vi "PathPlanner_Cmd_AutoHolonomicExecute.vi"(5 "PathPlanner_Cmd_FollowHolConfig":T17={"HOLONOMIC_CTRL_PACK_TUNING"={"X PID Tuning"={"Kp"=0.0, "Ki"=0.0, "Kd"=0.0, "MaximumIntegral"=9.9e+30, "MinimumIntegral"=-9.9e+30, "IntegralZone"=9.9e+30}, "Y PID Tuning"={"Kp"=0.0, "Ki"=0.0, "Kd"=0.0, "MaximumIntegral"=9.9e+30, "MinimumIntegral"=-9.9e+30, "IntegralZone"=9.9e+30}, "thetaProfiledPID_CTRL"={"Controller"={"Kp"=0.0, "Ki"=0.0, "Kd"=0.0, "Period"=0.0, "Max_Integral"=1.0, "Min_Integral"=-1.0, "Max_Input"=0.0, "Min_Input"=0.0, "Continuous"=FALSE, "PositionError"=0.0, "VelocityError"=0.0, "PrevError"=0.0, "Total_Integral"=0.0, "PositionTolerance"=0.05, "VelocityTolerance"=9.99e+35, "SetPoint"=0.0, "Kf"=0.0, "Prev_Deriv"=0.0, "Prev_Deriv 2"=0.0, "DerivativeFilter"=FALSE, "Min_Output"=-9.99e+35, "Max_Output"=9.9e+35, "Prev_F_P"=0.0, "Prev_F_P_2"=0.0, "AntiWindupActive"=FALSE, "Measurement"=0.0, "IntegralZone"=9.9e+30}, "Goal"={"Position"=0.0, "Velocity"=0.0}, "Setpoint"={"Position"=0.0, "Velocity"=0.0}, "Constraint"={"MaxVelocity"=0.0, "MaxAcceleration"=0.0}}}, "Max Wheel Speed M/S"=0.0, "Tolerance SI"={"TRANSLATION"={"X"=0.04, "Y"=0.04}, "ROTATION"={"VALUE"=0.034906585039887, "COS"=0.999390827019096, "SIN"=0.034899496702501}}, "Drive Base Radius M"=0.0, "ControlPastEnd_Sec"=3.0, "Period_Sec"=0.02, "Trigger Events"=TRUE} {"Tolerance SI"."ROTATION"."SIN" format="%13.4f"; "Tolerance SI"."ROTATION"."COS" format="%13.4f"; "Tolerance SI"."ROTATION"."VALUE" format="%13.4f"; "Tolerance SI"."TRANSLATION"."Y" format="%14.3f"; "Tolerance SI"."TRANSLATION"."X" format="%14.3f"; "HOLONOMIC_CTRL_PACK_TUNING"."thetaProfiledPID_CTRL"."Constraint"."MaxAcceleration" format="%16_6e"; "HOLONOMIC_CTRL_PACK_TUNING"."thetaProfiledPID_CTRL"."Constraint"."MaxVelocity" format="%16_6e"; "HOLONOMIC_CTRL_PACK_TUNING"."thetaProfiledPID_CTRL"."Setpoint"."Velocity" format="%16_6e"; "HOLONOMIC_CTRL_PACK_TUNING"."thetaProfiledPID_CTRL"."Setpoint"."Position" format="%16_6e"; "HOLONOMIC_CTRL_PACK_TUNING"."thetaProfiledPID_CTRL"."Goal"."Velocity" format="%16_6e"; "HOLONOMIC_CTRL_PACK_TUNING"."thetaProfiledPID_CTRL"."Goal"."Position" format="%16_6e"; "HOLONOMIC_CTRL_PACK_TUNING"."thetaProfiledPID_CTRL"."Controller"."IntegralZone" format="%16_6e"; "HOLONOMIC_CTRL_PACK_TUNING"."thetaProfiledPID_CTRL"."Controller"."Measurement" format="%16_6e"; "HOLONOMIC_CTRL_PACK_TUNING"."thetaProfiledPID_CTRL"."Controller"."Prev_F_P_2" format="%16_6e"; "HOLONOMIC_CTRL_PACK_TUNING"."thetaProfiledPID_CTRL"."Controller"."Prev_F_P" format="%16_6e"; "HOLONOMIC_CTRL_PACK_TUNING"."thetaProfiledPID_CTRL"."Controller"."Max_Output" format="%16_6e"; "HOLONOMIC_CTRL_PACK_TUNING"."thetaProfiledPID_CTRL"."Controller"."Min_Output" format="%16_6e"; "HOLONOMIC_CTRL_PACK_TUNING"."thetaProfiledPID_CTRL"."Controller"."Prev_Deriv 2" format="%16_6e"; "HOLONOMIC_CTRL_PACK_TUNING"."thetaProfiledPID_CTRL"."Controller"."Prev_Deriv" format="%16_6e"; "HOLONOMIC_CTRL_PACK_TUNING"."thetaProfiledPID_CTRL"."Controller"."Kf" format="%16_6e"; "HOLONOMIC_CTRL_PACK_TUNING"."thetaProfiledPID_CTRL"."Controller"."SetPoint" format="%16_6e"; "HOLONOMIC_CTRL_PACK_TUNING"."thetaProfiledPID_CTRL"."Controller"."VelocityTolerance" format="%16_6e"; "HOLONOMIC_CTRL_PACK_TUNING"."thetaProfiledPID_CTRL"."Controller"."PositionTolerance" format="%16_6e"; "HOLONOMIC_CTRL_PACK_TUNING"."thetaProfiledPID_CTRL"."Controller"."Total_Integral" format="%16_6e"; "HOLONOMIC_CTRL_PACK_TUNING"."thetaProfiledPID_CTRL"."Controller"."PrevError" format="%16_6e"; "HOLONOMIC_CTRL_PACK_TUNING"."thetaProfiledPID_CTRL"."Controller"."VelocityError" format="%16_6e"; "HOLONOMIC_CTRL_PACK_TUNING"."thetaProfiledPID_CTRL"."Controller"."PositionError" format="%16_6e"; "HOLONOMIC_CTRL_PACK_TUNING"."thetaProfiledPID_CTRL"."Controller"."Min_Input" format="%16_6e"; "HOLONOMIC_CTRL_PACK_TUNING"."thetaProfiledPID_CTRL"."Controller"."Max_Input" format="%16_6e"; "HOLONOMIC_CTRL_PACK_TUNING"."thetaProfiledPID_CTRL"."Controller"."Min_Integral" format="%16_6e"; "HOLONOMIC_CTRL_PACK_TUNING"."thetaProfiledPID_CTRL"."Controller"."Max_Integral" format="%16_6e"; "HOLONOMIC_CTRL_PACK_TUNING"."thetaProfiledPID_CTRL"."Controller"."Period" format="%16_6e"; "HOLONOMIC_CTRL_PACK_TUNING"."thetaProfiledPID_CTRL"."Controller"."Kd" format="%16_6e"; "HOLONOMIC_CTRL_PACK_TUNING"."thetaProfiledPID_CTRL"."Controller"."Ki" format="%16_6e"; "HOLONOMIC_CTRL_PACK_TUNING"."thetaProfiledPID_CTRL"."Controller"."Kp" format="%16_6e"}, 6 "PassthroughTime_SEC":dbl=-1.0, 7 "PathPlanner_Cmd_AutoConfig":T2 {"Paths"."IdealStartingState"."Rotation"."SIN" format="%13.4f"; "Paths"."IdealStartingState"."Rotation"."COS" format="%13.4f"; "Paths"."IdealStartingState"."Rotation"."VALUE" format="%13.4f"; "Paths"."PointTowardsZones"."TargetPosition"."Y" format="%14.3f"; "Paths"."PointTowardsZones"."TargetPosition"."X" format="%14.3f"; "Paths"."PointTowardsZones"."RotationOffset"."SIN" format="%13.4f"; "Paths"."PointTowardsZones"."RotationOffset"."COS" format="%13.4f"; "Paths"."PointTowardsZones"."RotationOffset"."VALUE" format="%13.4f"; "Paths"."Waypoints"."nextControl"."Y" format="%14.3f"; "Paths"."Waypoints"."nextControl"."X" format="%14.3f"; "Paths"."Waypoints"."anchor"."Y" format="%14.3f"; "Paths"."Waypoints"."anchor"."X" format="%14.3f"; "Paths"."Waypoints"."prevControl"."Y" format="%14.3f"; "Paths"."Waypoints"."prevControl"."X" format="%14.3f"; "Paths"."AllPoints"."RotationTarget"."rotation"."SIN" format="%13.4f"; "Paths"."AllPoints"."RotationTarget"."rotation"."COS" format="%13.4f"; "Paths"."AllPoints"."RotationTarget"."rotation"."VALUE" format="%13.4f"; "Paths"."AllPoints"."Position"."Y" format="%14.3f"; "Paths"."AllPoints"."Position"."X" format="%14.3f"; "Paths"."GoalEndState"."Rotation"."SIN" format="%13.4f"; "Paths"."GoalEndState"."Rotation"."COS" format="%13.4f"; "Paths"."GoalEndState"."Rotation"."VALUE" format="%13.4f"; "Paths"."RotationTargets"."rotation"."SIN" format="%13.4f"; "Paths"."RotationTargets"."rotation"."COS" format="%13.4f"; "Paths"."RotationTargets"."rotation"."VALUE" format="%13.4f"}, 8 "Enabled":bool=TRUE, 9 "Reset":bool, 10 "CurrentChassisSpeeds":T1 {"vOmega" format="%10.3f"; "vY" format="%10.3f"; "vX" format="%10.3f"}, 11 "Current Pose SI":T24={"TRANSLATION"={"X"=0.0, "Y"=0.0}, "ROTATION"={"VALUE"=0.0, "COS"=1.0, "SIN"=0.0}} {"ROTATION"."SIN" format="%13.4f"; "ROTATION"."COS" format="%13.4f"; "ROTATION"."VALUE" format="%13.4f"; "TRANSLATION"."Y" format="%14.3f"; "TRANSLATION"."X" format="%14.3f"}) -> (0 "Position Error M":dbl, 1 "Complete":bool, 2 "At Reference":bool, 3 "calcChassisSpeed":T1 {"vOmega" format="%10.3f"; "vY" format="%10.3f"; "vX" format="%10.3f"})   [LabVIEW 2019, in "PathPlanner24.lvlib"]
doc: "DOCUMENTATION IS NOT COMPLETE.\n \nCalculates the next output of the path following controller for holonomic drive robots. This wraps a Holonomic Drive Control function with the particulars needed to follow a PathPlanner trajectory.\n\nInputs:\n - PathPlanner_Holonomic_Ctrl_Pack_Tuning - cluster - The tuning paraameters for the holonomic drive controller. These are static. They should not be changed after the first call to this function.\n - CurrentPoseSi - pose2d - The current pose calculated by odometry or pose estimation. The pose can be absolute or relative depending on what type of trajectory is being followed.\n - PathPlannerState - cluster - The path palnner trajectory state containing the desired position and velocities of the robot.\n - Reset - boolean - When TRUE the holonomic drive controller is reset. This should be set to TRUE for the first execution of a trajectory.\n - Enabled - boolean - When TRUE, closed loop control is enabled. (Optional. Default: TRUE)\n - Period - double - The loop period in seconds for this controller. (Optional. Default: 0.020)\n\nOutputs:\n - CalcChassisSpeed - cluster - The desired chassis speed in SI units.\n - AtReference - boolean - TRUE if the robots position is within the defined tolerance.\n - PositionError - pose2d - Position error in SI units. How far the robot is away from the desired trajectory position.\n - out_Holonomic_Drive_Ctrl - THe current holonomic drive controller data cluster. This is mainly for diagnostic purposes."
uses:
  PathPlanner24.lvlib
  <vilib>/Rock Robotics/WPI/ThirdParty/JAS_Junk/TrajLib/TypeDef/CHASSIS_SPEEDS.ctl
  <vilib>/Rock Robotics/WPI/ThirdParty/JAS_Junk/TrajLib/Trajectory_Library.lvlib
  <vilib>/Rock Robotics/WPI/ThirdParty/JAS_Junk/TrajLib/TypeDef/TRANSLATION2D.ctl
  <vilib>/Rock Robotics/WPI/ThirdParty/JAS_Junk/TrajLib/TypeDef/ROTATION2D.ctl
  <vilib>/Rock Robotics/WPI/ThirdParty/JAS_Junk/TrajLib/TypeDef/POSE2D.ctl
  <vilib>/Rock Robotics/WPI/ThirdParty/JAS_Junk/TrajLib/TypeDef/PID_TUNING.ctl
  <vilib>/Rock Robotics/WPI/ThirdParty/JAS_Junk/TrajLib/TypeDef/PID_CONTROLLER.ctl
  <vilib>/Rock Robotics/WPI/ThirdParty/JAS_Junk/TrajLib/TypeDef/TRAPEZOID_PROFILE_STATE.ctl
  <vilib>/Rock Robotics/WPI/ThirdParty/JAS_Junk/TrajLib/TypeDef/TRAPEZOID_PROFILE_CONSTRAINT.ctl
  <vilib>/Rock Robotics/WPI/ThirdParty/JAS_Junk/TrajLib/TypeDef/PROFILED_PID_CONTROLLER.ctl
  <vilib>/Rock Robotics/WPI/ThirdParty/JAS_Junk/TrajLib/TypeDef/HOLONOMIC_PACK_TUNING.ctl
  TypeDef/PathPlannerRotationTarget.ctl
  TypeDef/PathPlannerPathConstraints.ctl
  TypeDef/PathPlannerConstraintsZone.ctl
  TypeDef/PathPlannerCommandUtil.ctl
  TypeDef/PathPlannerEventMarker.ctl
  TypeDef/PathPlannerGoalEndState.ctl
  TypeDef/PathPlannerPathPoint.ctl
  TypeDef/PathPlannerPath.ctl
  TypeDef/PathPlannerCmdFollowHolConfig.ctl
  TypeDef/PathPlannerWaypoint.ctl
  TypeDef/PathPlannerPointTowardsZone.ctl
  TypeDef/PathPlannerIdealStartingState.ctl
  TypeDef/PathPlannerCmdPathPlannerAutoConfig.ctl
  ENum/PathPlanner_CommandUtil_Type_ENUM.ctl
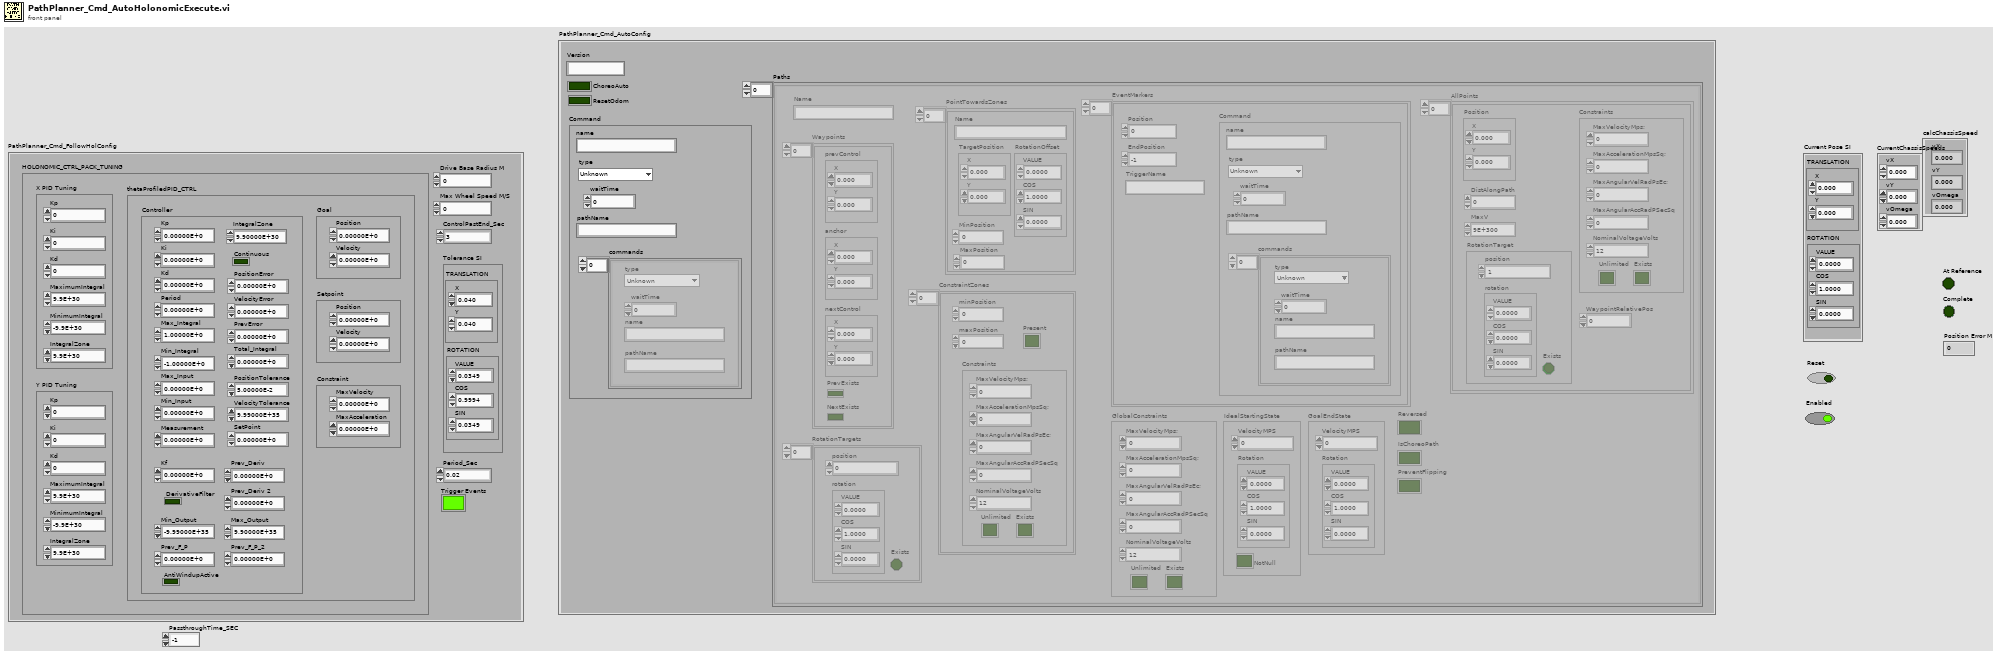
[diagram p1: front panel]
types:
  T1 = typedef "Trajectory_Library.lvlib/CHASSIS_SPEEDS.ctl" = cluster{"vX":dbl, "vY":dbl, "vOmega":dbl}
  T2 = typedef "PathPlanner24.lvlib/PathPlannerCmdPathPlannerAutoConfig.ctl" = cluster{"Command":T3, "ChoreoAuto":bool, "Version":string, "ResetOdom":bool, "Paths":T5[]}
  T3 = typedef "PathPlanner24.lvlib/PathPlannerCommandUtil.ctl" = cluster{"waitTime":dbl, "name":string, "pathName":string, "commands":cluster{"type":T4, "waitTime":dbl, "name":string, "pathName":string}[], "type":T4}
  T4 = typedef "PathPlanner24.lvlib/PathPlanner_CommandUtil_Type_ENUM.ctl" = enum16{"Unknown", "Wait", "Named", "Path", "Sequential", "Parallel", "Race", "Deadline", "PointTowardsZoneEnter", "PointTowardsZoneExit", "TriggerEventStart", "TriggerEventStop", "TriggerEventOneshot"}
  T5 = typedef "PathPlanner24.lvlib/PathPlannerPath.ctl" = cluster{"Reversed":bool, "RotationTargets":T6[], "ConstraintZones":T8[], "EventMarkers":T10[], "GlobalConstraints":T9, "GoalEndState":T11, "AllPoints":T12[], "Name":string, "Waypoints":T14[], "PointTowardsZones":T15[], "IdealStartingState":T16, "IsChoreoPath":bool, "PreventFlipping":bool}
  T6 = typedef "PathPlanner24.lvlib/PathPlannerRotationTarget.ctl" = cluster{"position":dbl, "rotation":T7, "Exists":bool}
  T7 = typedef "Trajectory_Library.lvlib/ROTATION2D.ctl" = cluster{"VALUE":dbl, "COS":dbl, "SIN":dbl}
  T8 = typedef "PathPlanner24.lvlib/PathPlannerConstraintsZone.ctl" = cluster{"minPosition":dbl, "maxPosition":dbl, "Constraints":T9, "Present":bool}
  T9 = typedef "PathPlanner24.lvlib/PathPlannerPathConstraints.ctl" = cluster{"MaxVelocityMps;":dbl, "MaxAccelerationMpsSq;":dbl, "MaxAngularVelRadPsEc;":dbl, "MaxAngularAccRadPSecSq":dbl, "Exists":bool, "Unlimited":bool, "NominalVoltageVolts":dbl}
  T10 = typedef "PathPlanner24.lvlib/PathPlannerEventMarker.ctl" = cluster{"Position":dbl, "Command":T3, "TriggerName":string, "EndPosition":dbl}
  T11 = typedef "PathPlanner24.lvlib/PathPlannerGoalEndState.ctl" = cluster{"VelocityMPS":dbl, "Rotation":T7}
  T12 = typedef "PathPlanner24.lvlib/PathPlannerPathPoint.ctl" = cluster{"Position":T13, "DistAlongPath":dbl, "MaxV":dbl, "Constraints":T9, "RotationTarget":T6, "WaypointRelativePos":dbl}
  T13 = typedef "Trajectory_Library.lvlib/TRANSLATION2D.ctl" = cluster{"X":dbl, "Y":dbl}
  T14 = typedef "PathPlanner24.lvlib/PathPlannerWaypoint.ctl" = cluster{"prevControl":T13, "anchor":T13, "nextControl":T13, "PrevExists":bool, "NextExists":bool}
  T15 = typedef "PathPlanner24.lvlib/PathPlannerPointTowardsZone.ctl" = cluster{"RotationOffset":T7, "Name":string, "TargetPosition":T13, "MinPosition":dbl, "MaxPosition":dbl}
  T16 = typedef "PathPlanner24.lvlib/PathPlannerIdealStartingState.ctl" = cluster{"VelocityMPS":dbl, "Rotation":T7, "NotNull":bool}
  T17 = typedef "PathPlanner24.lvlib/PathPlannerCmdFollowHolConfig.ctl" = cluster{"HOLONOMIC_CTRL_PACK_TUNING":T18, "Max Wheel Speed M/S":dbl, "Tolerance SI":T24, "Drive Base Radius M":dbl, "ControlPastEnd_Sec":dbl, "Period_Sec":dbl, "Trigger Events":bool}
  T18 = typedef "Trajectory_Library.lvlib/HOLONOMIC_PACK_TUNING.ctl" = cluster{"X PID Tuning":T19, "Y PID Tuning":T19, "thetaProfiledPID_CTRL":T20}
  T19 = typedef "Trajectory_Library.lvlib/PID_TUNING.ctl" = cluster{"Kp":dbl, "Ki":dbl, "Kd":dbl, "MaximumIntegral":dbl, "MinimumIntegral":dbl, "IntegralZone":dbl}
  T20 = typedef "Trajectory_Library.lvlib/PROFILED_PID_CONTROLLER.ctl" = cluster{"Controller":T21, "Goal":T22, "Setpoint":T22, "Constraint":T23}
  T21 = typedef "Trajectory_Library.lvlib/PID_CONTROLLER.ctl" = cluster{"Kp":dbl, "Ki":dbl, "Kd":dbl, "Period":dbl, "Max_Integral":dbl, "Min_Integral":dbl, "Max_Input":dbl, "Min_Input":dbl, "Continuous":bool, "PositionError":dbl, "VelocityError":dbl, "PrevError":dbl, "Total_Integral":dbl, "PositionTolerance":dbl, "VelocityTolerance":dbl, "SetPoint":dbl, "Kf":dbl, "Prev_Deriv":dbl, "Prev_Deriv 2":dbl, "DerivativeFilter":bool, "Min_Output":dbl, "Max_Output":dbl, "Prev_F_P":dbl, "Prev_F_P_2":dbl, "AntiWindupActive":bool, "Measurement":dbl, "IntegralZone":dbl}
  T22 = typedef "Trajectory_Library.lvlib/TRAPEZOID_PROFILE_STATE.ctl" = cluster{"Position":dbl, "Velocity":dbl}
  T23 = typedef "Trajectory_Library.lvlib/TRAPEZOID_PROFILE_CONSTRAINT.ctl" = cluster{"MaxVelocity":dbl, "MaxAcceleration":dbl}
  T24 = typedef "Trajectory_Library.lvlib/POSE2D.ctl" = cluster{"TRANSLATION":T13, "ROTATION":T7}
  T25 = cluster{"type":T4, "waitTime":dbl, "name":string, "pathName":string}[]
  T26 = cluster{"type":T4, "waitTime":dbl, "name":string, "pathName":string}
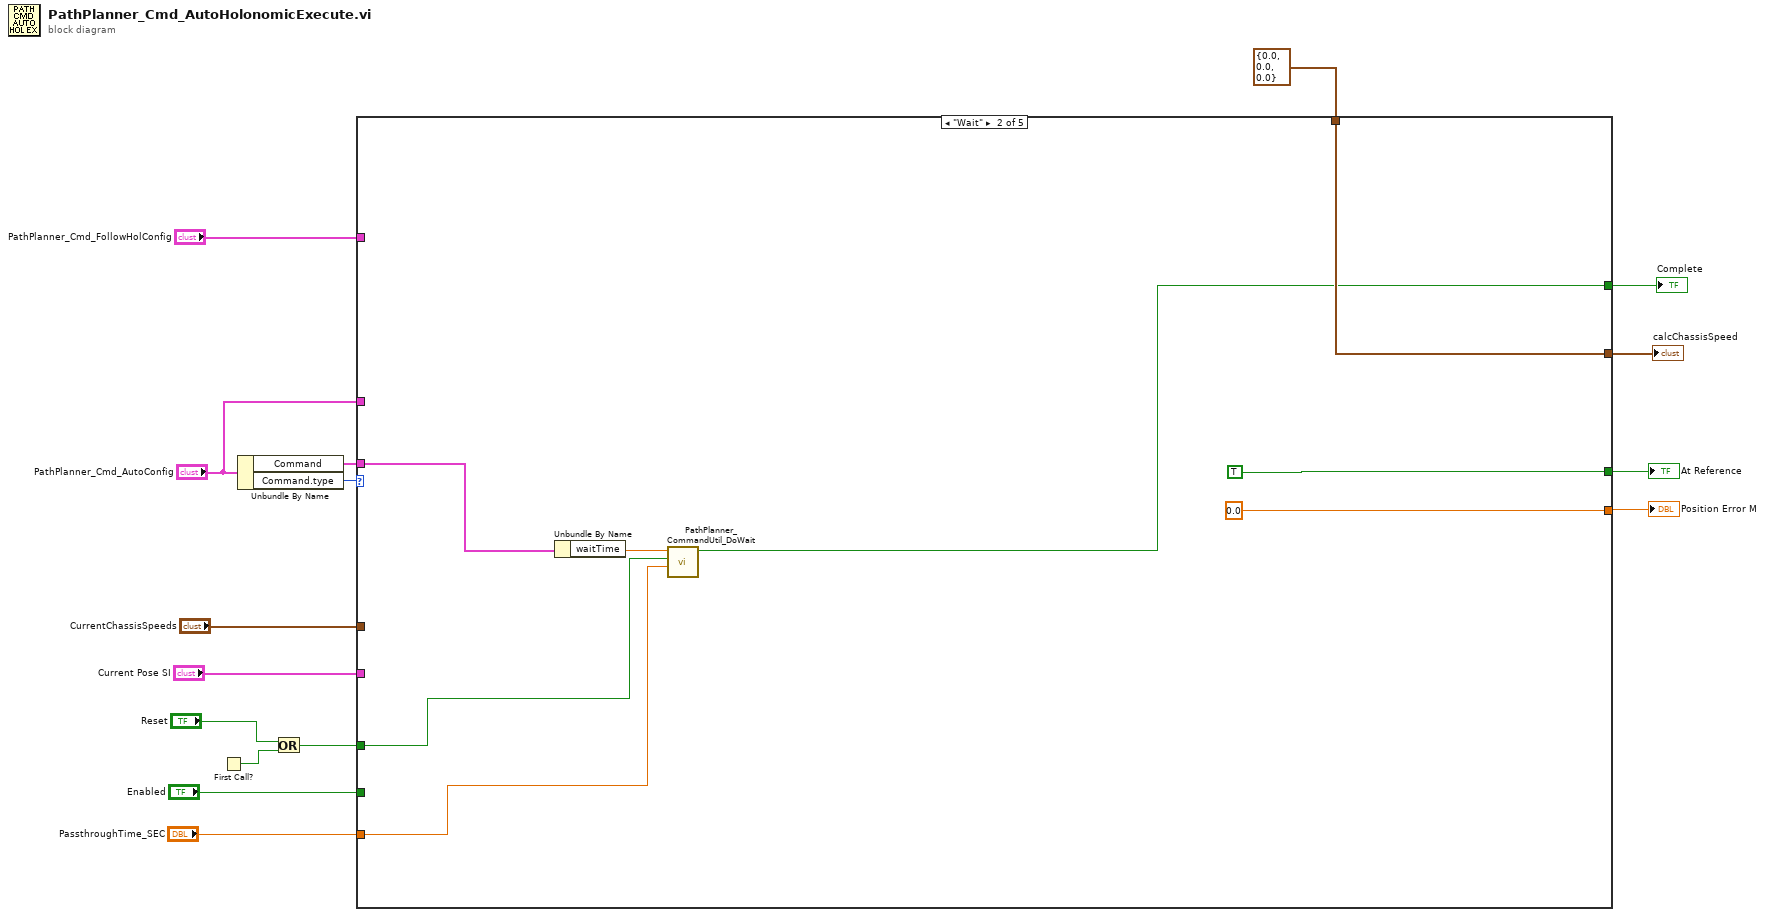
[diagram p0: block diagram]
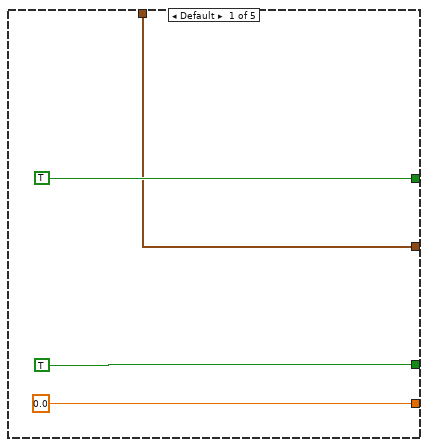
[diagram p2: hidden frame]
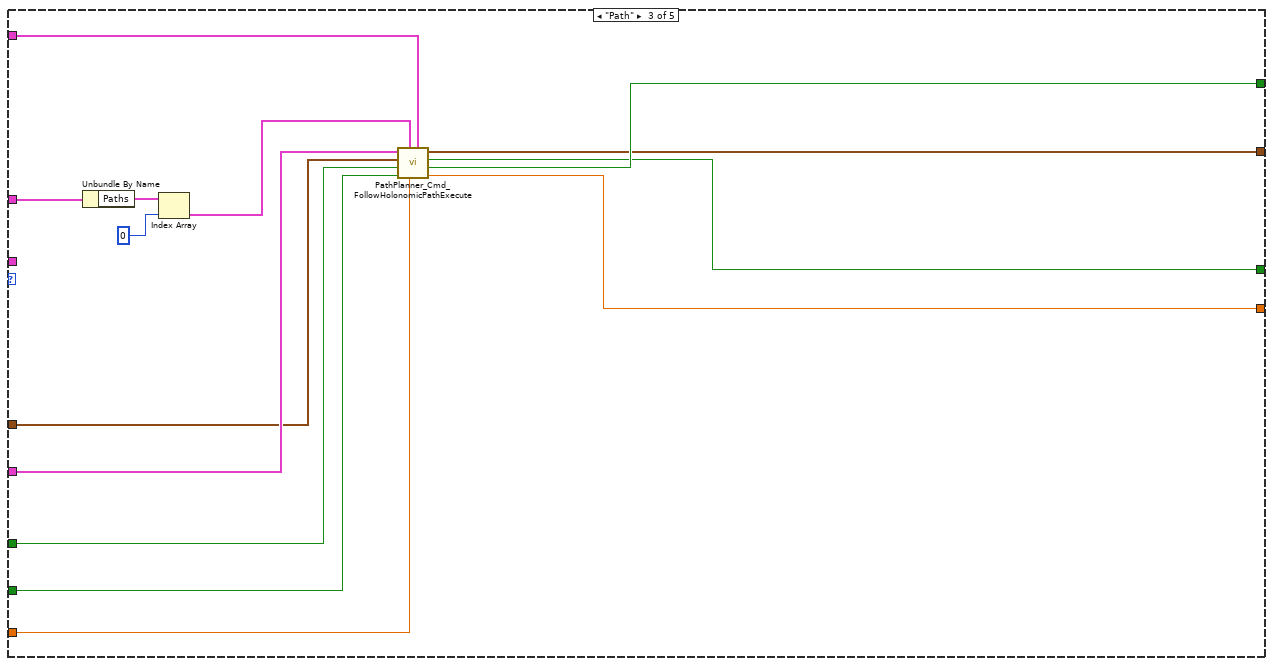
[diagram p3: hidden frame]
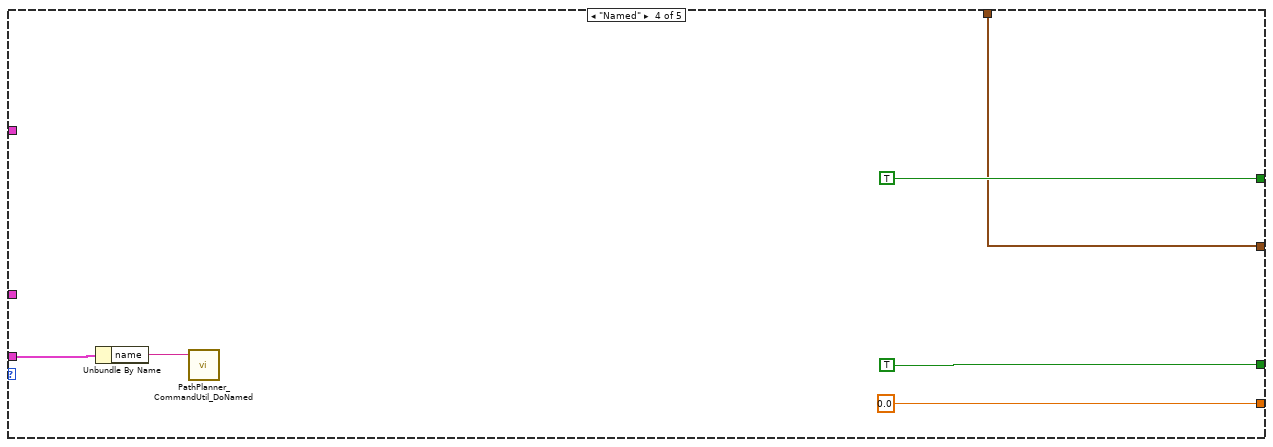
[diagram p4: hidden frame]
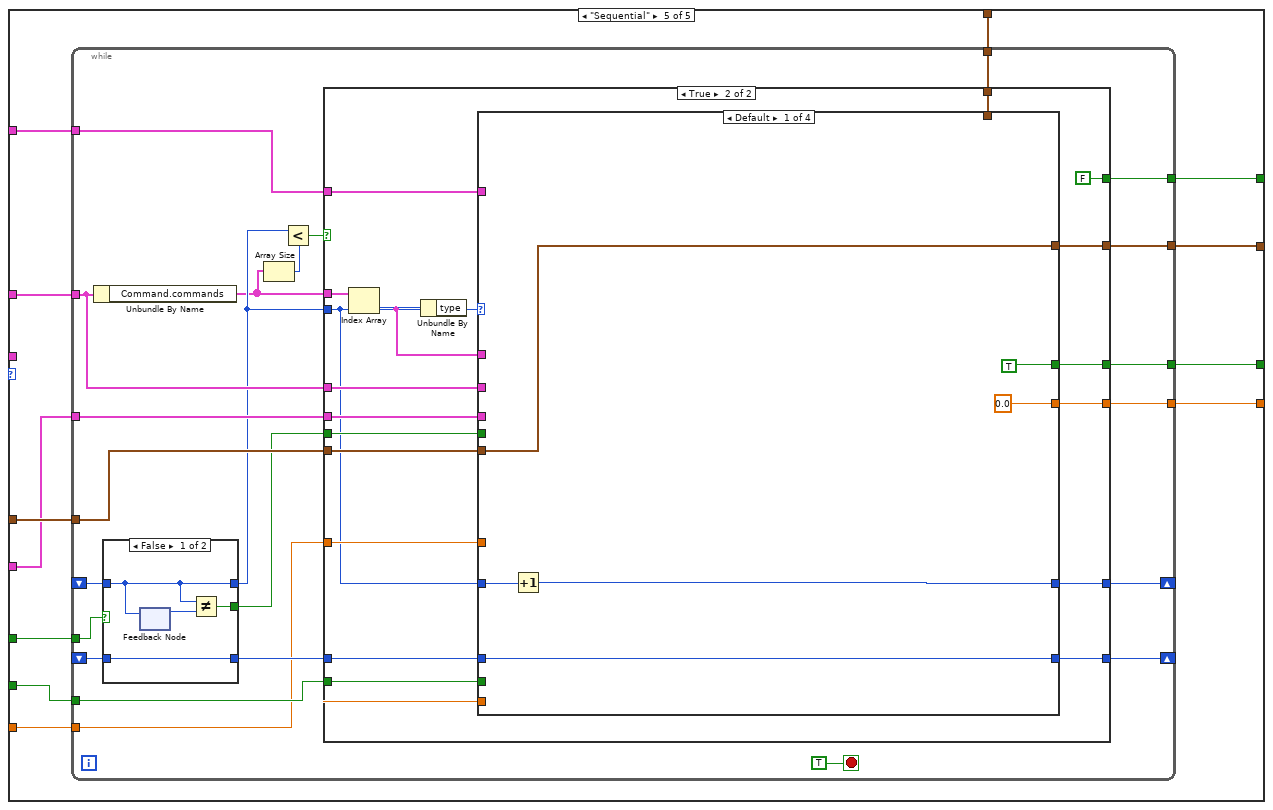
[diagram p5: hidden frame]
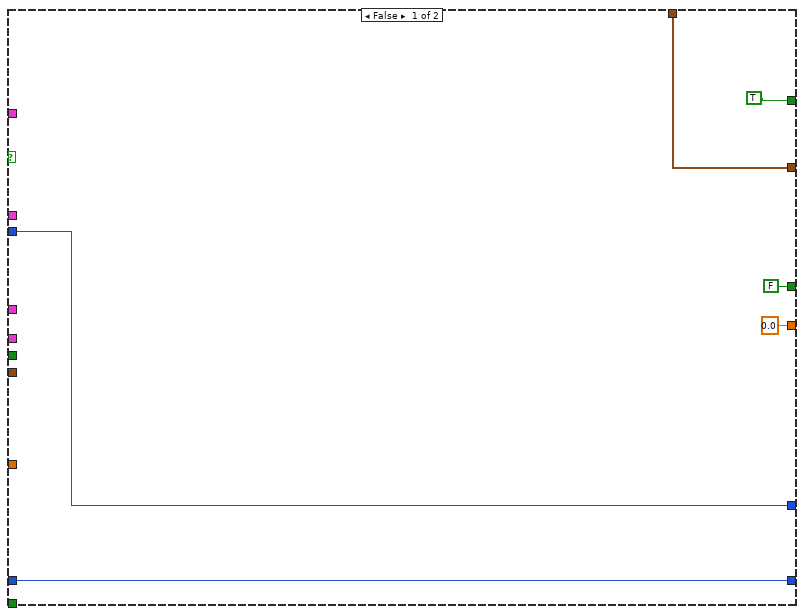
[diagram p6: hidden frame]
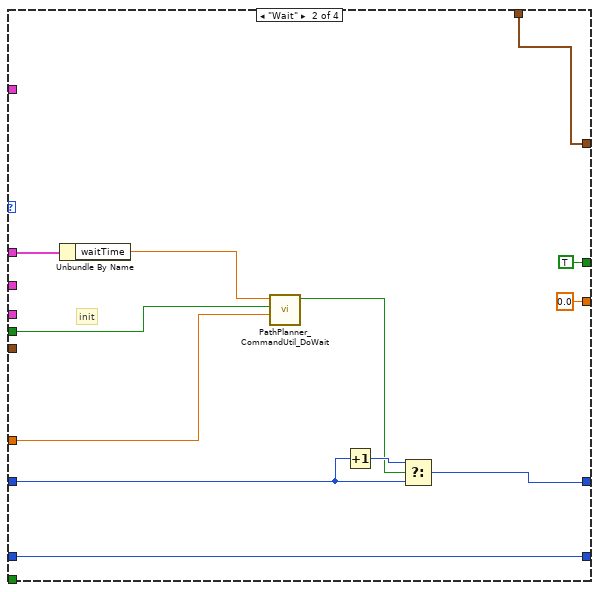
[diagram p7: hidden frame]
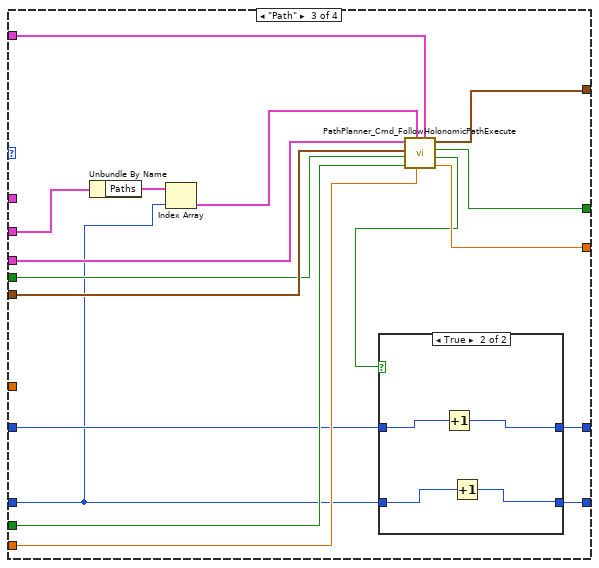
[diagram p8: hidden frame]
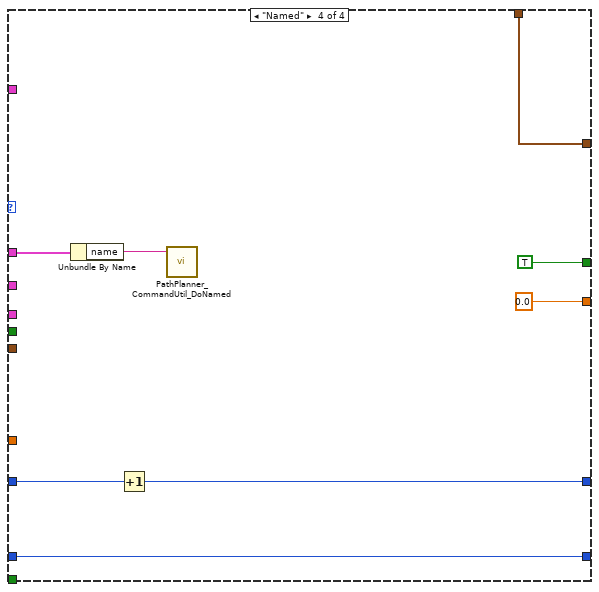
[diagram p10: hidden frame]
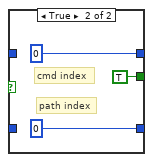
[diagram p11: hidden frame]
diagram:
  n1 = First Call?() -> (First Call?: T/F=w15:bool)
  n2 = Unbundle By Name("PathPlanner_Cmd_AutoConfig") -> ("Command"=w13:T3, "Command.type"=w14:T4)
  n3 = Or(x="Reset", y=w15) -> (x .or. y?=w8:bool)
  n4 = case shown="\"Wait\"" w14 {
    tunnel: w13 -> [_ w24 _ w44 _]
    tunnel: "PathPlanner_Cmd_AutoConfig" -> [_ _ w42 _ w59]
    tunnel: "PathPlanner_Cmd_FollowHolConfig" -> [_ _ w38 _ w52]
    tunnel: "Current Pose SI" -> [_ _ w37 _ w51]
    tunnel: "CurrentChassisSpeeds" -> [_ _ w36 _ w58]
    tunnel: w8 -> [_ w23 w35 _ w60]
    tunnel: "Enabled" -> [_ _ w34 _ w50]
    tunnel: "PassthroughTime_SEC" -> [_ w22 w33 _ w54]
    tunnel: [0.0 ("Position Error M") 0.0 ("Position Error M") w32 0.0 ("Position Error M") w55] -> w5
    tunnel: [TRUE ("Complete") w21 w31 TRUE ("Complete") w49] -> w4
    tunnel: [TRUE ("At Reference") TRUE ("At Reference") w30 TRUE ("At Reference") w56] -> w3
    tunnel: [w17 w26 w29 w45 w57] -> w2
    tunnel: T1 {"vX"=0.0, "vY"=0.0, "vOmega"=0.0} ("CurrentChassisSpeeds") -> [w17 w26 _ w45 w53]
    frame Default {
    }
    frame "Wait" {
      n5 = Unbundle By Name(w24) -> ("waitTime"=w25:dbl)
      n6 = call "PathPlanner_CommandUtil_DoWait.vi"("PassthroughTime_SEC"=w22, "Init"=w23, "WaitTimeSec"=w25) -> ("Done"=w21:bool)  [unwired: 8 in]
    }
    frame "Path" {
      n7 = Unbundle By Name(w42) -> ("Paths"=w41:T5[])
      n8 = Index Array(array=w41, index=0) -> (element=w39:T5)
      n9 = call "PathPlanner_Cmd_FollowHolonomicPathExecute.vi"("PathPlanner_Cmd_FollowHolConfig"=w38, "PassthroughTime_SEC"=w33, "PathPlannerPath"=w39, "Enabled"=w34, "Reset"=w35, "CurrentChassisSpeeds"=w36, "Current Pose SI"=w37) -> ("Position Error M"=w32:dbl, "Complete"=w31:bool, "At Reference"=w30:bool, "calcChassisSpeed"=w29:T1)  [unwired: 1 out]
    }
    frame "Named" {
      n10 = Unbundle By Name(w44) -> ("name"=w43:string)
      n11 = call "PathPlanner_CommandUtil_DoNamed.vi"("Event Action Name"=w43) -> ()  [unwired: 11 in]
    }
    frame "Sequential" {
      n12 = while {
        tunnel: w60 -> [w78]
        tunnel: w59 -> [w73]
        tunnel: w58 -> [w82]
        tunnel: [w81] -> w57
        tunnel: [w80] -> w56
        tunnel: [w79] -> w55
        tunnel: w54 -> [w68]
        shift-right: [w67] -> _
        shift-left: _ -> [w77]
        shift-right: [w66] -> _
        shift-left: _ -> [w76]
        tunnel: w53 -> [w74]
        tunnel: w52 -> [w71]
        tunnel: w51 -> [w70]
        tunnel: w50 -> [w69]
        tunnel: [w61] -> w49
        stop <- TRUE stop-if-true
        n13 = Unbundle By Name(w73) -> ("Command.commands"=w63:T25)
        n14 = case shown="False" w78 {
          tunnel: [w158 0] -> w65
          tunnel: [w160 0] -> w72
          tunnel: w77 -> [w158 _]
          tunnel: w76 -> [w160 _]
          tunnel: [w161 TRUE] -> w75
          frame False {
            n15 = feedback-in #1(w158) -> ()
            n16 = feedback #1() -> (w159:i32)  [unwired: 1 in]
            n17 = Not Equal?(x=w158, y=w159) -> (x != y?=w161:bool)
          }
          frame True {
            # "path index"
            # "cmd index"
          }
        }
        n18 = Array Size(array=w63) -> (size(s)=w64:i32)
        n19 = Less?(x=w65, y=w64) -> (x < y?=w62:bool)
        n20 = case shown="True" w62 {
          tunnel: w82 -> [_ w108]
          tunnel: [w88 w107] -> w81
          tunnel: [FALSE ("At Reference") w106] -> w80
          tunnel: [0.0 ("Position Error M") w105] -> w79
          tunnel: w63 -> [_ w104]
          tunnel: w75 -> [_ w102]
          tunnel: w74 -> [w88 w100]
          tunnel: w73 -> [_ w99]
          tunnel: w72 -> [w84 w98]
          tunnel: w71 -> [_ w97]
          tunnel: w70 -> [_ w96]
          tunnel: w69 -> [_ w95]
          tunnel: w68 -> [_ w94]
          tunnel: w65 -> [w85 w90]
          tunnel: [w85 w93] -> w67
          tunnel: [w84 w92] -> w66
          tunnel: [TRUE FALSE] -> w61
          frame False {
          }
          frame True {
            n21 = Index Array(array=w104, index=w90) -> (element=w101:T26)
            n22 = Unbundle By Name(w101) -> ("type"=w103:T4)
            n23 = case shown="Default" w103 {
              tunnel: w108 -> [w114 _ w138 _]
              tunnel: [w114 w124 w134 w156] -> w107
              tunnel: [TRUE TRUE ("At Reference") w133 TRUE ("At Reference")] -> w106
              tunnel: [0.0 0.0 ("Position Error M") w132 0.0 ("Position Error M")] -> w105
              tunnel: w94 -> [_ w126 _ _]
              tunnel: w102 -> [_ w125 w137 _]
              tunnel: w101 -> [_ w120 _ w157]
              tunnel: w100 -> [_ w124 _ w156]
              tunnel: w99 -> [_ _ w141 _]
              tunnel: w98 -> [w109 w123 w129 w151]
              tunnel: w97 -> [_ _ w140 _]
              tunnel: w96 -> [_ _ w139 _]
              tunnel: w95 -> [_ _ w136 _]
              tunnel: w94 -> [_ _ w135 _]
              tunnel: w90 -> [w111 w116 w130 w153]
              tunnel: [w110 w115 w127 w152] -> w93
              tunnel: [w109 w123 w128 w151] -> w92
              frame Default {
                n24 = Increment(x=w111) -> (x+1=w110:i32)
              }
              frame "Wait" {
                # "init"
                n25 = Unbundle By Name(w120) -> ("waitTime"=w119:dbl)
                n26 = call "PathPlanner_CommandUtil_DoWait.vi"("PassthroughTime_SEC"=w126, "Init"=w125, "WaitTimeSec"=w119) -> ("Done"=w117:bool)  [unwired: 8 in]
                n27 = Increment(x=w116) -> (x+1=w118:i32)
                n28 = Select(t=w118, s=w117, f=w116) -> (s? t:f=w115:i32)
              }
              frame "Path" {
                n29 = Unbundle By Name(w141) -> ("Paths"=w143:T5[])
                n30 = Index Array(array=w143, index=w129) -> (element=w142:T5)
                n31 = call "PathPlanner_Cmd_FollowHolonomicPathExecute.vi"("PathPlanner_Cmd_FollowHolConfig"=w140, "PassthroughTime_SEC"=w135, "PathPlannerPath"=w142, "Enabled"=w136, "Reset"=w137, "CurrentChassisSpeeds"=w138, "Current Pose SI"=w139) -> ("Position Error M"=w132:dbl, "Complete"=w131:bool, "At Reference"=w133:bool, "calcChassisSpeed"=w134:T1)  [unwired: 1 out]
                n32 = case shown="True" w131 {
                  tunnel: w130 -> [w144 w149]
                  tunnel: w129 -> [w145 w147]
                  tunnel: [w145 w146] -> w128
                  tunnel: [w144 w148] -> w127
                  frame False {
                  }
                  frame True {
                    n33 = Increment(x=w149) -> (x+1=w148:i32)
                    n34 = Increment(x=w147) -> (x+1=w146:i32)
                  }
                }
              }
              frame "Named" {
                n35 = Unbundle By Name(w157) -> ("name"=w150:string)
                n36 = Increment(x=w153) -> (x+1=w152:i32)
                n37 = call "PathPlanner_CommandUtil_DoNamed.vi"("Event Action Name"=w150) -> ()  [unwired: 11 in]
              }
            }
          }
        }
      }
    }
  }
  "At Reference" <- w3
  "Position Error M" <- w5
  "calcChassisSpeed" <- w2
  "Complete" <- w4
